vi "Initialize.vi"(7 "Project Store in":refnum<class "Project Store-INI.lvclass">, 8 "error in (no error)":errorcluster, 11 "Data Folder":path) -> (0 "error out":errorcluster, 5 "Project Store out":refnum<class "Project Store-INI.lvclass">)   [LabVIEW 2024, in "Project Store-INI.lvclass"]
doc: "Remembers the data folder that holds Projects.ini and Tasks.ini. Call it before Read from Data Source and Write to Data Source. Nothing is read or written here.\n\nGenerated by: Claude"
uses:
  Project Store-INI.lvclass
  Project Store-INI.lvclass/Project Store-INI.ctl
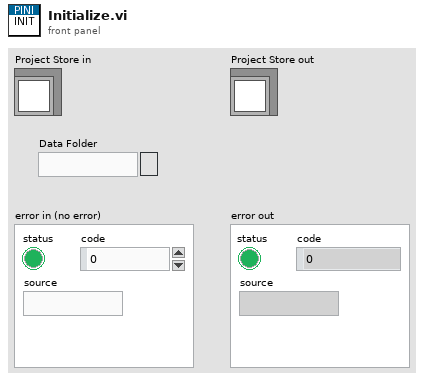
[diagram p1: front panel]
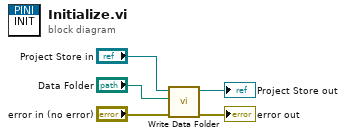
[diagram p0: block diagram]
diagram:
  n1 = call-dynamic "Write Data Folder.vi"("error in (no error)"="error in (no error)", "Data Folder"="Data Folder", "Project Store-INI in"="Project Store in") -> ("error out"=→"error out":errorcluster, "Project Store-INI out"=→"Project Store out":refnum<class "Project Store-INI.lvclass">)  [unwired: 7 in]
